vi "DO seq.vi"(0 "Channel Names":string[](array[string])=["DO00", "DO01", "DO02", "DO03", "DO04", "DO05", "DO06", "DO07", "DO08", "DO09", "DO10", "DO11", "DO12", "DO13", "DO14", "DO15", "DO16", "DO17", "DO18", "DO19", "DO20", "DO21", "DO22", "DO23", "DO24", "DO25", "DO26", "DO27", "DO28", "DO29", "DO30", "DO31", "DO32", "DO33", "DO34", "DO35", "DO36", "DO37", "DO38", "DO39", "DO40", "DO41", "DO42", "DO43", "DO44", "DO45", "DO46", "DO47", "DO48", "DO49", "DO50", "DO51", "DO52", "DO53", "DO54", "DO55", "DO56", "DO57", "DO58", "DO59", "DO60", "DO61", "DO62", "DO63"], 5 "Sequence Table":string[][](array[string])=[["DO01", "1", "5"], ["DO63", "3", "8"]]) -> (4 "DO Output":bool[](array[boolean]), 6 "Time (s)":dbl)   [LabVIEW 2026]
doc: "시퀀스 테이블 기반 DO 출력 시험 VI (상태머신 구조: Idle / Init / Run / Exit).\n[Idle] 대기. 시험 시작 -> Init, 종료 -> Exit.\n[Init] 시퀀스 테이블 1열의 채널 이름을 Channel Names 배열에서 검색해 인덱스를 구하고(0부터 시작, DO01=1), 2열 On Time / 3열 Off Time(초)을 숫자로 변환. DO Output 전부 OFF, Time=0, 시작 시각 기록 -> Run.\n[Run] 50 ms마다 경과 시간 갱신, 각 행 채널을 On Time <= Time < Off Time 동안 ON. Time이 가장 큰 Off Time에 도달(>=)하거나 시험 정지를 누르면 -> Idle (출력 유지), 시험 시작을 다시 누르면 -> Init(초기화 후 재시작).\n[Exit] 루프 종료.\n같은 채널이 여러 행에 있으면 아래쪽 행의 판정이 우선한다. 테이블에 없는 채널 이름은 무시된다."
panel:
  in  "Exit":bool
  in  "Stop":bool
  in  "Start":bool
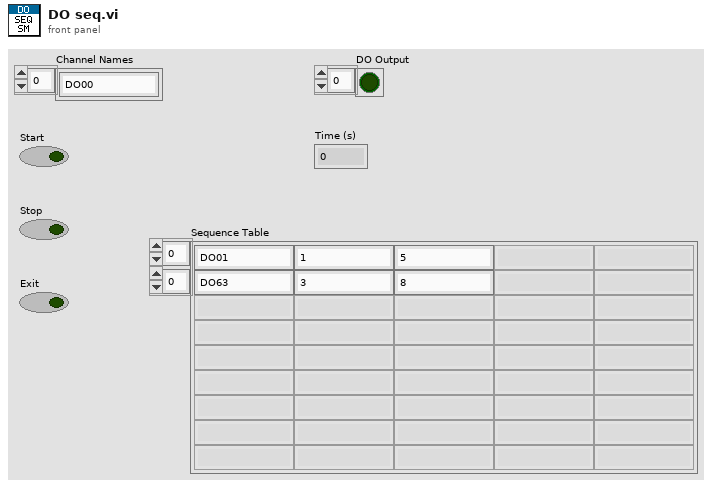
[diagram p1: front panel]
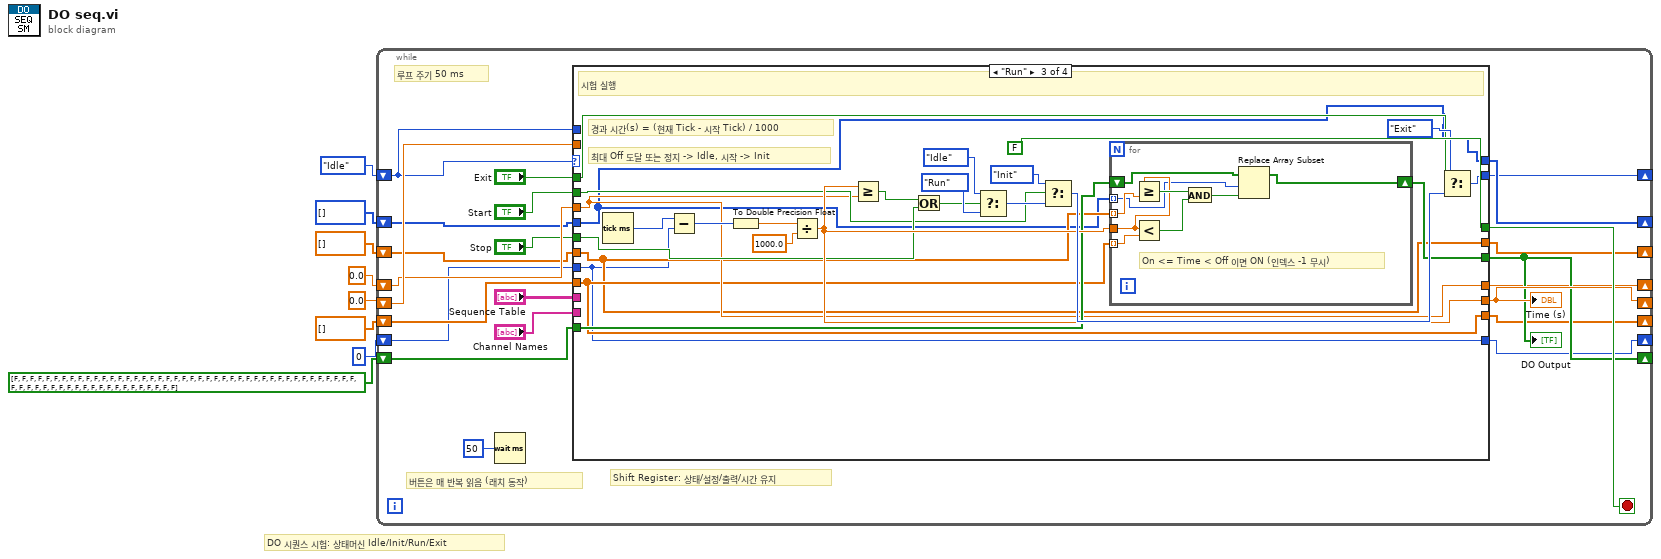
[diagram p0: block diagram]
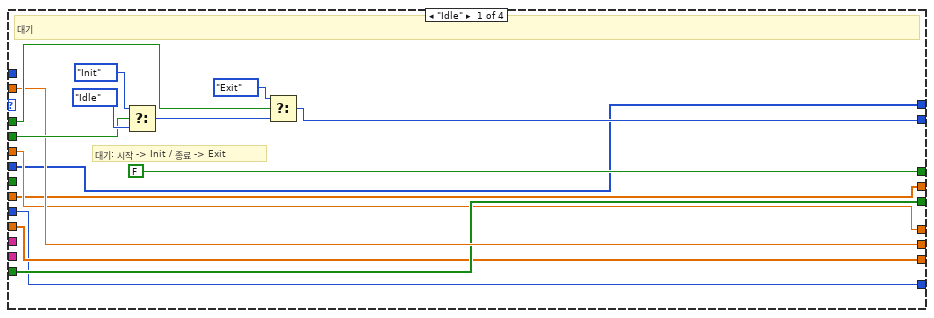
[diagram p2: hidden frame]
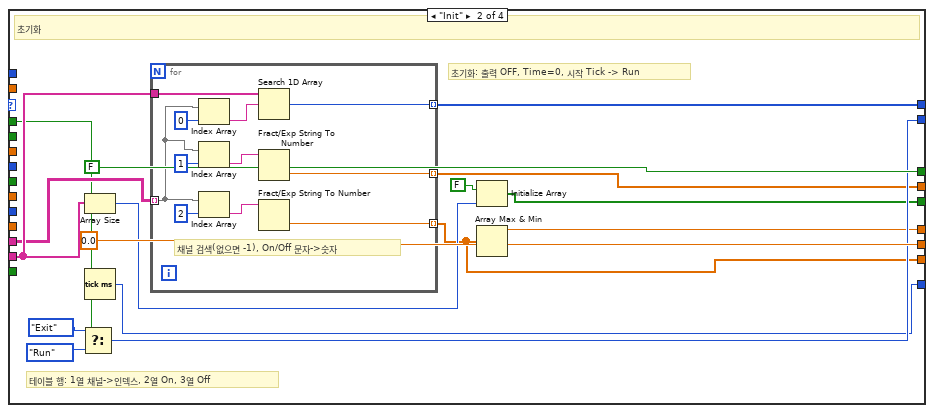
[diagram p3: hidden frame]
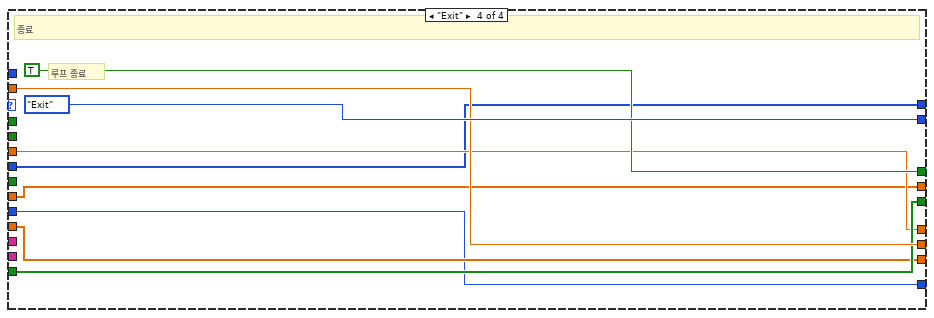
[diagram p4: hidden frame]
diagram:
  # "DO 시퀀스 시험: 상태머신 Idle/Init/Run/Exit"
  n1 = while {
    shift-right: [w23] -> _
    shift-left: enum16{"Idle", "Init", "Run", "Exit"}."Idle" -> [w15]
    shift-right: [w24] -> _
    shift-left: u32 0 -> [w16]
    shift-right: [w25] -> _
    shift-left: i32[] [] -> [w17]
    shift-right: [w26] -> _
    shift-left: dbl[] [] -> [w18]
    shift-right: [w27] -> _
    shift-left: dbl[] [] -> [w19]
    shift-right: [w28] -> _
    shift-left: 0.0 -> [w20]
    shift-right: [w29] -> _
    shift-left: bool[] [FALSE, FALSE, FALSE, FALSE, FALSE, FALSE, FALSE, FALSE, FALSE, FALSE, FALSE, FALSE, FALSE, FALSE, FALSE, FALSE, FALSE, FALSE, FALSE, FALSE, FALSE, FALSE, FALSE, FALSE, FALSE, FALSE, FALSE, FALSE, FALSE, FALSE, FALSE, FALSE, FALSE, FALSE, FALSE, FALSE, FALSE, FALSE, FALSE, FALSE, FALSE, FALSE, FALSE, FALSE, FALSE, FALSE, FALSE, FALSE, FALSE, FALSE, FALSE, FALSE, FALSE, FALSE, FALSE, FALSE, FALSE, FALSE, FALSE, FALSE, FALSE, FALSE, FALSE, FALSE] -> [w21]
    shift-right: [w30] -> _
    shift-left: 0.0 -> [w22]
    stop <- w31 stop-if-true
    # "Shift Register: 상태/설정/출력/시간 유지"
    # "루프 주기 50 ms"
    # "버튼은 매 반복 읽음 (래치 동작)"
    n2 = Wait (ms)(milliseconds to wait=u32 50) -> ()  [unwired: 1 out]
    n3 = case shown="\"Run\"" w15 {
      tunnel: "Start" -> [w39 _ w80 _]
      tunnel: "Stop" -> [_ _ w81 _]
      tunnel: "Exit" -> [w40 w47 w82 _]
      tunnel: "Sequence Table" -> [_ w48 _ _]
      tunnel: "Channel Names" -> [_ w49 _ _]
      tunnel: [FALSE FALSE FALSE TRUE] -> w31
      tunnel: w15 -> [_ _ _ _]
      tunnel: w16 -> [w32 _ w74 w108]
      tunnel: w17 -> [w33 _ w75 w109]
      tunnel: w18 -> [w34 _ w76 w110]
      tunnel: w19 -> [w35 _ w77 w111]
      tunnel: w20 -> [w36 _ w78 w112]
      tunnel: w21 -> [w37 _ w79 w113]
      tunnel: w22 -> [w38 _ _ w114]
      tunnel: [w32 w57 w74 w108] -> w24
      tunnel: [w33 w50 w75 w109] -> w25
      tunnel: [w34 w51 w76 w110] -> w26
      tunnel: [w35 w52 w77 w111] -> w27
      tunnel: [w36 w53 w78 w112] -> w28
      tunnel: [w37 w56 w88 w113] -> w29
      tunnel: [w38 0.0 w87 w114] -> w30
      tunnel: [w45 w60 w97 enum16{"Idle", "Init", "Run", "Exit"}."Exit"] -> w23
      frame "Idle" {
        # "대기: 시작 -> Init / 종료 -> Exit"
        # "대기"
        n4 = Select(t=enum16{"Idle", "Init", "Run", "Exit"}."Init", s=w39, f=enum16{"Idle", "Init", "Run", "Exit"}."Idle") -> (s? t:f=w43:enum16{"Idle", "Init", "Run", "Exit"})
        n5 = Select(t=enum16{"Idle", "Init", "Run", "Exit"}."Exit", s=w40, f=w43) -> (s? t:f=w45:enum16{"Idle", "Init", "Run", "Exit"})
      }
      frame "Init" {
        # "초기화: 출력 OFF, Time=0, 시작 Tick -> Run"
        # "테이블 행: 1열 채널->인덱스, 2열 On, 3열 Off"
        # "초기화"
        n6 = Select(t=enum16{"Idle", "Init", "Run", "Exit"}."Exit", s=w47, f=enum16{"Idle", "Init", "Run", "Exit"}."Run") -> (s? t:f=w60:enum16{"Idle", "Init", "Run", "Exit"})
        n7 = Array Size(array=w49) -> (size(s)=w54:i32)
        n8 = Tick Count (ms)() -> (millisecond timer value=w57:u32)
        n9 = for {
          tunnel: w48 -> [w63] mode=indexing
          tunnel: w49 -> [w64]
          tunnel: [w71] -> w50 mode=indexing
          tunnel: [w72] -> w51 mode=indexing
          tunnel: [w73] -> w52 mode=indexing
          # "채널 검색(없으면 -1), On/Off 문자->숫자"
          n10 = Index Array(array=w63, index=0) -> (element=w66:string)
          n11 = Index Array(array=w63, index=1) -> (element=w68:string)
          n12 = Index Array(array=w63, index=2) -> (element=w70:string)
          n13 = Search 1D Array(1D array=w64, element=w66) -> (index of element=w71:i32)  [unwired: 1 in]
          n14 = Fract/Exp String To Number(string=w68) -> (number=w72:dbl)  [unwired: 3 in, 1 out]
          n15 = Fract/Exp String To Number(string=w70) -> (number=w73:dbl)  [unwired: 3 in, 1 out]
        }
        n16 = Initialize Array(FALSE, w54) -> (w56:bool[])
        n17 = Array Max & Min(array=w52) -> (max value=w53:dbl)  [unwired: 3 out]
      }
      frame "Run" {
        # "최대 Off 도달 또는 정지 -> Idle, 시작 -> Init"
        # "경과 시간(s) = (현재 Tick - 시작 Tick) / 1000"
        # "시험 실행"
        n18 = Tick Count (ms)() -> (millisecond timer value=w83:u32)
        n19 = Subtract(x=w83, y=w74) -> (x-y=w84:u32)
        n20 = To Double Precision Float(number=w84) -> (double precision float=w85:dbl)
        n21 = Divide(x=w85, y=1000.0) -> (x/y=w87:dbl)
        n22 = Greater Or Equal?(x=w87, y=w78) -> (x >= y?=w89:bool)
        n23 = Or(x=w89, y=w81) -> (x .or. y?=w90:bool)
        n24 = Select(t=enum16{"Idle", "Init", "Run", "Exit"}."Idle", s=w90, f=enum16{"Idle", "Init", "Run", "Exit"}."Run") -> (s? t:f=w93:enum16{"Idle", "Init", "Run", "Exit"})
        n25 = Select(t=enum16{"Idle", "Init", "Run", "Exit"}."Init", s=w80, f=w93) -> (s? t:f=w95:enum16{"Idle", "Init", "Run", "Exit"})
        n26 = for {
          tunnel: w75 -> [w99] mode=indexing
          tunnel: w76 -> [w100] mode=indexing
          tunnel: w77 -> [w101] mode=indexing
          shift-right: [w106] -> w88
          shift-left: w79 -> [w107]
          tunnel: w87 -> [w102]
          # "On <= Time < Off 이면 ON (인덱스 -1 무시)"
          n27 = Greater Or Equal?(x=w102, y=w100) -> (x >= y?=w103:bool)
          n28 = Less?(x=w102, y=w101) -> (x < y?=w104:bool)
          n29 = And(x=w103, y=w104) -> (x .and. y?=w105:bool)
          n30 = Replace Array Subset(array=w107, new element=w105, index=w99) -> (w106:bool[])
        }
        n31 = Select(t=enum16{"Idle", "Init", "Run", "Exit"}."Exit", s=w82, f=w95) -> (s? t:f=w97:enum16{"Idle", "Init", "Run", "Exit"})
      }
      frame "Exit" {
        # "루프 종료"
        # "종료"
      }
    }
    "DO Output" <- w29
    "Time (s)" <- w30
  }
